vi "Day 13.vi"() -> ()   [LabVIEW 2021]
uses:
  <vilib>/Utility/file.llb/Read Delimited Spreadsheet (string).vi
  <vilib>/regexp/Match Regular Expression.xnode
panel:
  out "Array":bool[][](array[boolean])
  out "sum":i16
  out "subarray":string[](array[string])
  in  "Input File":enum32{"example input", "input"}(radio)
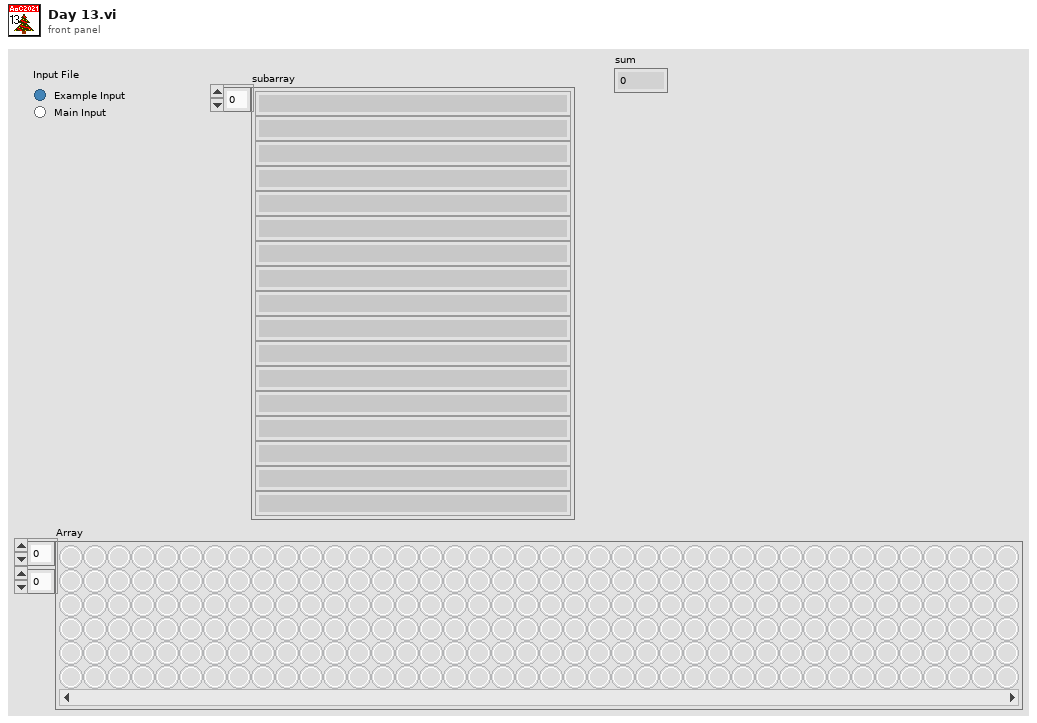
[diagram p1: front panel]
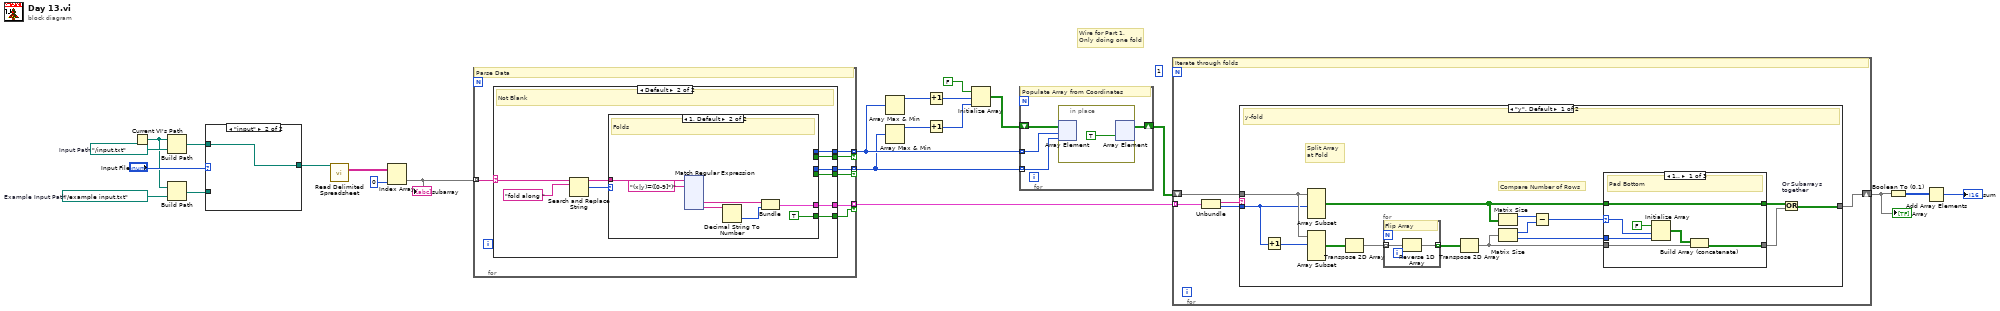
[diagram p0: block diagram]
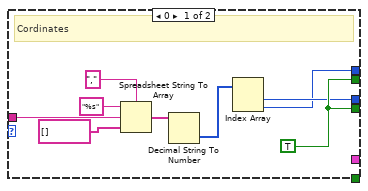
[diagram p3: hidden frame]
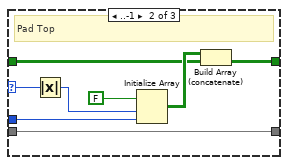
[diagram p5: hidden frame]
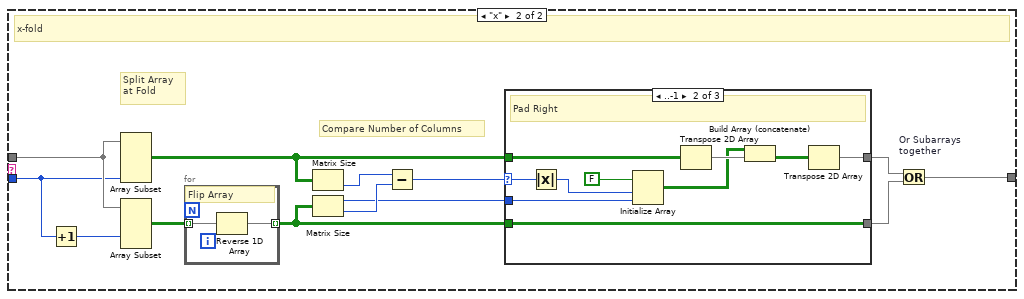
[diagram p7: hidden frame]
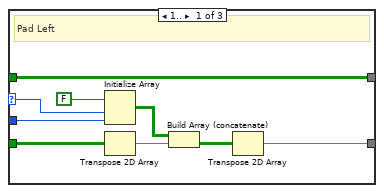
[diagram p8: hidden frame]
diagram:
  (unwired) 1
  w22 = path "../example input.txt"  # Example Input Path
  w23 = path "../input.txt"  # Input Path
  # "Wire for Part 1,\nOnly doing one fold"
  n1 = Current VI's Path() -> (path=w17:path)
  n2 = Build Path(base path=w17, name or relative path=w23) -> (appended path=w20:path)
  n3 = Build Path(base path=w17, name or relative path=w22) -> (appended path=w19:path)
  n4 = case shown="\"input\"" "Input File" {
    tunnel: w20 -> [_ w25]
    tunnel: w19 -> [w24 _]
    tunnel: [w24 w25] -> w18
    frame "example input" {
    }
    frame "input" {
    }
  }
  n5 = call-poly <vilib>:"Read Delimited Spreadsheet.vi"("file path (dialog if empty)"=w18) -> ("all rows"=w16:string[][])  [unwired: 9 in, 5 out]
  n6 = Index Array(array=w16, index (col)=0 ("disabled index (col)")) -> (element=w14:string[])  [unwired: 1 in]
  "subarray" <- w14
  n7 = for {
    tunnel: w14 -> [w32] mode=indexing
    tunnel: [w31] -> w13 mode=indexing if=w30
    tunnel: [w29] -> w5 mode=indexing if=w28
    tunnel: [w27] -> w12 mode=indexing if=w26
    # "Parse Data"
    n8 = case shown="Default" w32 {
      selector: w32 -> [_ w42]
      tunnel: [_ w38] -> w31
      tunnel: [_ w37] -> w30
      tunnel: [_ w36] -> w29
      tunnel: [_ w35] -> w28
      tunnel: [_ w34] -> w27
      tunnel: [_ w33] -> w26
      frame "" {
        # "Blank row"
      }
      frame Default {
        # "Not Blank"
        n9 = Search and Replace String(input string=w42, search string="fold along ") -> (result string=w39:string, number of replacements=w40:i32)  [unwired: 6 in, 2 out]
        n10 = case shown="1, Default" w40 {
          tunnel: w39 -> [w51 w58]
          tunnel: [w43 _] -> w38
          tunnel: [w45 _] -> w37
          tunnel: [_ w53] -> w36
          tunnel: [_ TRUE] -> w35
          tunnel: [w44 _] -> w34
          tunnel: [w45 _] -> w33
          frame 0 {
            w45 = TRUE
            # "Cordinates"
            n11 = Spreadsheet String To Array(delimiter (Tab)=",", format string="%s", spreadsheet string=w51, array type (2D Dbl)=string[] []) -> (array=w47:string[])
            n12 = Decimal String To Number(string=w47) -> (number=w46:i32[])  [unwired: 2 in, 1 out]
            n13 = Index Array(array=w46) -> (element #1=w44:i32, element #2=w43:i32)  [unwired: 2 in]
          }
          frame 1, Default {
            # "Folds"
            n14 = xnode "Match Regular Expression"("input string"=w58, "regular expression"="(x|y)=([0-9]*)") -> ("submatch 1"=w55:string, "submatch 2"=w56:string)  [unwired: 4 in, 5 out]
            n15 = Decimal String To Number(string=w56) -> (number=w54:i32)  [unwired: 2 in, 1 out]
            n16 = Bundle("submatch 1"=w55, w54) -> (w53:cluster{"submatch 1":string, i32})  [unwired: 1 in]
          }
        }
      }
    }
  }
  n17 = Array Max & Min(array=w13) -> (max value=w11:i32)  [unwired: 3 out]
  n18 = Array Max & Min(array=w12) -> (max value=w8:i32)  [unwired: 3 out]
  n19 = Increment(x=w11) -> (x+1=w9:i32)
  n20 = Increment(x=w8) -> (x+1=w7:i32)
  n21 = Initialize Array(FALSE, w9, w7) -> (w6:bool[][])
  n22 = for {
    tunnel: w13 -> [w181] mode=indexing
    tunnel: w12 -> [w180] mode=indexing
    shift-right: [w179] -> w4
    shift-left: w6 -> [w182]
    # "Populate Array from Coordinates"
    n23 = in-place {
      n24 = in-place-array #1(w182, w181, w180) -> ()  [unwired: 1 out]
      n25 = in-place-array #1(TRUE) -> (w179:bool[][])  [unwired: 2 out]
    }
  }
  n26 = for {
    tunnel: w5 -> [w188] mode=indexing
    shift-right: [w184] -> w3
    shift-left: w4 -> [w185]
    # "Iterate through folds"
    n27 = Unbundle(w188) -> ("submatch 1"=w187:string, w186:i32)
    n28 = case shown="\"y\", Default" w187 {
      tunnel: w186 -> [w201 w228]
      tunnel: w185 -> [w203 w235]
      tunnel: [w194 w233] -> w184
      frame "y", Default {
        # "Compare Number of Rows"
        # "Split Array at Fold"
        # "y-fold"
        n29 = Increment(x=w201) -> (x+1=w200:i32)
        n30 = Array Subset(array=w203, length (row)=w201) -> (w192:bool[][])  [unwired: 3 in]
        n31 = Array Subset(array=w203, index (row)=w200) -> (w202:bool[][])  [unwired: 3 in]
        n32 = Transpose 2D Array(2D array=w202) -> (transposed array=w199:bool[][])
        n33 = for {
          tunnel: w199 -> [w222] mode=indexing
          tunnel: [w221] -> w198 mode=indexing
          # "Flip Array"
          n34 = Reverse 1D Array(array=w222) -> (reversed array=w221:bool[])
        }
        n35 = Transpose 2D Array(2D array=w198) -> (transposed array=w190:bool[][])
        n36 = Matrix Size(0:w192) -> (1:w197:i32)  [unwired: 1 out]
        n37 = Matrix Size(0:w190) -> (1:w196:i32, 2:w189:i32)
        n38 = Subtract(x=w197, y=w196) -> (x-y=w195:i32)
        n39 = case shown="1.." w195 {
          selector: w195 -> [w209 w217 _]
          tunnel: [w204 w214 w220] -> w193
          tunnel: w192 -> [w204 w213 w220]
          tunnel: [w205 w212 w219] -> w191
          tunnel: w190 -> [w206 w212 w219]
          tunnel: w189 -> [w208 w216 _]
          frame 1.. {
            # "Pad Bottom"
            n40 = Initialize Array(FALSE, w209, w208) -> (w207:bool[][])
            n41 = Build Array (concatenate)(w207, w206) -> (w205:bool[][])
          }
          frame ..-1 {
            # "Pad Top"
            n42 = Absolute Value(x=w217) -> (abs(x)=w211:i32)
            n43 = Initialize Array(FALSE, w211, w216) -> (w215:bool[][])
            n44 = Build Array (concatenate)(w215, w213) -> (w214:bool[][])
          }
          frame 0 {
            # "Same Size"
          }
        }
        n45 = Or "Or Subarrays\ntogether"(x=w193, y=w191) -> (x .or. y?=w194:bool[][])
      }
      frame "x" {
        # "Compare Number of Columns"
        # "Split Array at Fold"
        # "x-fold"
        n46 = Increment(x=w228) -> (x+1=w229:i32)
        n47 = Array Subset(array=w235, length (col)=w228) -> (w231:bool[][])  [unwired: 3 in]
        n48 = Array Subset(array=w235, index (col)=w229) -> (w227:bool[][])  [unwired: 3 in]
        n49 = for {
          tunnel: w227 -> [w258] mode=indexing
          tunnel: [w257] -> w226 mode=indexing
          # "Flip Array"
          n50 = Reverse 1D Array(array=w258) -> (reversed array=w257:bool[])
        }
        n51 = Matrix Size(0:w231) -> (2:w225:i32)  [unwired: 1 out]
        n52 = Matrix Size(0:w226) -> (1:w223:i32, 2:w224:i32)
        n53 = Subtract(x=w225, y=w224) -> (x-y=w234:i32)
        n54 = case shown="..-1" w234 {
          selector: w234 -> [w241 w251 _]
          tunnel: [w243 w247 w256] -> w232
          tunnel: w231 -> [w243 w253 w256]
          tunnel: [w236 w252 w255] -> w230
          tunnel: w226 -> [w237 w252 w255]
          tunnel: w223 -> [w240 w245 _]
          frame 1.. {
            # "Pad Left"
            n55 = Initialize Array(FALSE, w241, w240) -> (w238:bool[][])
            n56 = Transpose 2D Array(2D array=w237) -> (transposed array=w239:bool[][])
            n57 = Build Array (concatenate)(w238, w239) -> (w242:bool[][])
            n58 = Transpose 2D Array(2D array=w242) -> (transposed array=w236:bool[][])
          }
          frame ..-1 {
            # "Pad Right"
            n59 = Absolute Value(x=w251) -> (abs(x)=w246:i32)
            n60 = Initialize Array(FALSE, w246, w245) -> (w249:bool[][])
            n61 = Transpose 2D Array(2D array=w253) -> (transposed array=w250:bool[][])
            n62 = Build Array (concatenate)(w249, w250) -> (w248:bool[][])
            n63 = Transpose 2D Array(2D array=w248) -> (transposed array=w247:bool[][])
          }
          frame 0 {
            # "Same Size"
          }
        }
        n64 = Or "Or Subarrays\ntogether"(x=w232, y=w230) -> (x .or. y?=w233:bool[][])
      }
    }
  }
  "Array" <- w3
  n65 = Boolean To (0,1)(Boolean=w3) -> (0, 1=w2:i16[][])
  n66 = Add Array Elements(numeric array=w2) -> (sum=→"sum":i16)
